vi "Simple SFTP File Download.vi"() -> ()   [LabVIEW 2018]
doc: "Downloads, or receives, a relatively small file from a remote SFTP server. This is similar to the SFTP command line utility when transferring, or copying, a remote file to a local destination. If performance is poor or memory is limited on the local machine, then it could be because the file is relatively large and this implementation is not very efficient for relatively large files."
uses:
  Toolkit/Session/Support/Create from SSH.vi
  Toolkit/Session/Support/Password Authentication.vi
  Toolkit/SFTP/Support/Create from Session.vi
  Toolkit/SFTP File/Support/Open from SFTP.vi
  Toolkit/SFTP File/Support/Close to SFTP.vi
  Toolkit/SFTP/Support/Destroy to Session.vi
  Toolkit/Session/Support/Destroy to SSH.vi
  Toolkit/SSH/SSH.lvclass
  Toolkit/Session/Session.lvclass
  Toolkit/SFTP/SFTP.lvclass
  Toolkit/SFTP File/SFTP File.lvclass
panel:
  in  "Remote File":string
  in  "Local File":path
  in  "Remote SFTP Server":string
  in  "Password":string
  in  "Username":string
  # "Overview: Demonstrates transferring, or downloading, a remote file from a SSH server, similar to the SFTP command line utility\nInstructions:\n1. Enter the IP address or host name of the remote SFTP server. This can be a CompactRIO (cRIO) running the National Instruments Linux Real-Time (NI Linux RT) operating system with the Enable Secure Shell Server (sshd) checkbox checked. \n2. Enter a username. If using a cRIO with a default configuration, then the username is \"admin\".\n3. Enter a password for the username. If using a cRIO with a default configuration, then the password is blank (empty).\n4. Enter the path and/or filename of the remote file to download. Typically, this is a POSIX/UNIX file path with a backslash, \"/\", used to separate directories and the default directory is the remote user's home directory, i.e. \"/home/admin\" on a default configured cRIO.\n5. Select a destination on the local computer for the transfer/download from the remote SSH server.\n6. Run this VI."
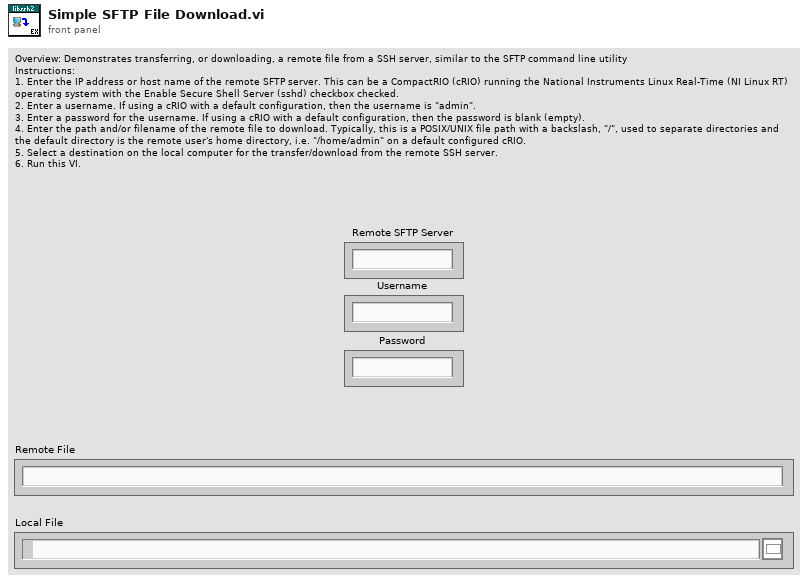
[diagram p1: front panel]
types:
  T1 = enum16{"open", "replace", "create", "open or create", "replace or create", "replace or create with confirmation"}
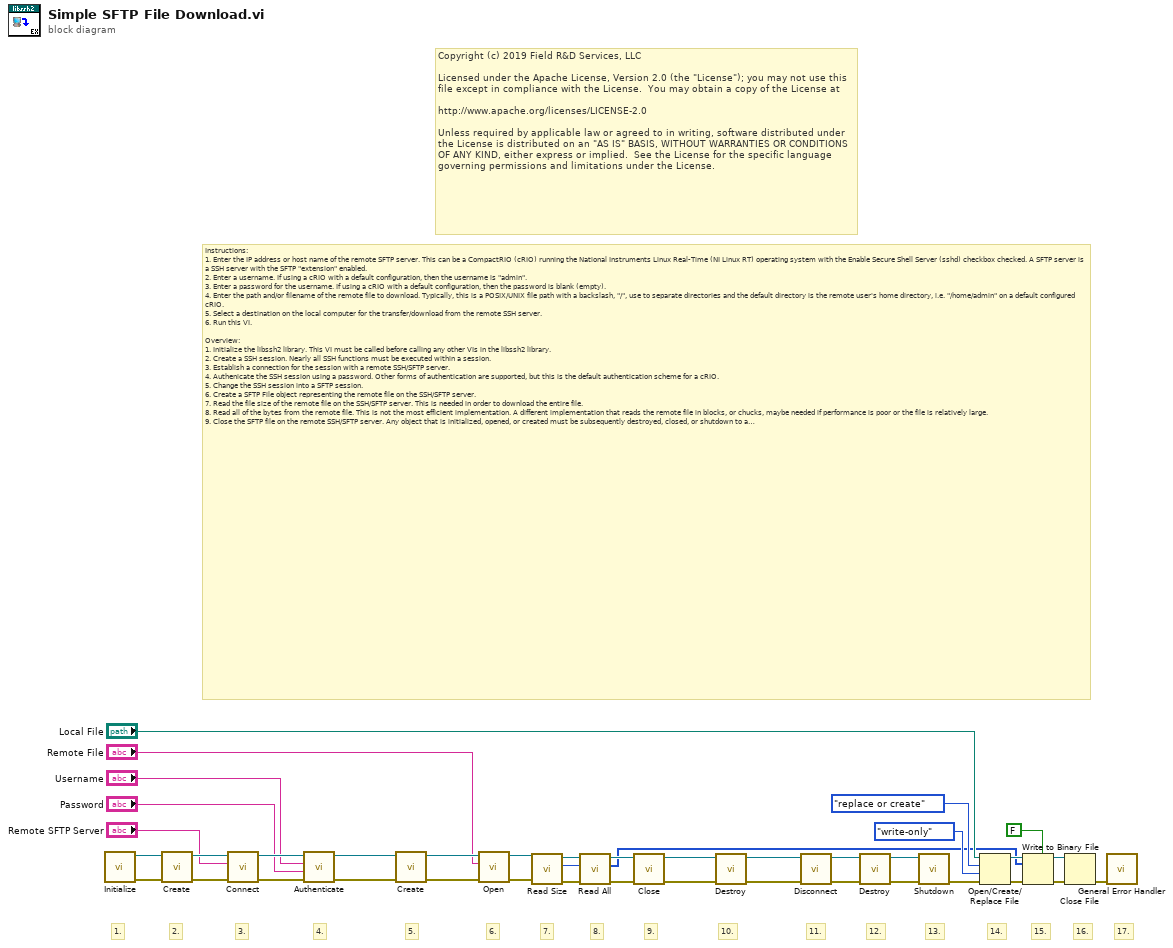
[diagram p0: block diagram]
diagram:
  # "8."
  # "17."
  # "16."
  # "Copyright (c) 2019 Field R&D Services, LLC\n\nLicensed under the Apache License, Version 2.0 (the \"License\"); you may not use this file except in compliance with the License.  You may obtain a copy of the License at\n\nhttp://www.apache.org/licenses/LICENSE-2.0\n\nUnless required by applicable law or agreed to in writing, software distributed under the License is distributed on an \"AS IS\" BASIS, WITHOUT WARRANTIES OR CONDITIONS OF ANY KIND, either express or implied.  See the License for the specific language governing permissions and limitations under the License."
  # "15."
  # "14."
  # "13."
  # "12."
  # "11."
  # "10."
  # "9."
  # "7."
  # "6."
  # "5."
  # "4."
  # "3."
  # "2."
  # "1."
  # "Instructions:\n1. Enter the IP address or host name of the remote SFTP server. This can be a CompactRIO (cRIO) running the National Instruments Linux Real-Time (NI Linux RT) operating system with the Enable Secure Shell Server (sshd) checkbox checked. A SFTP server is a SSH server with the SFTP \"extension\" enabled.\n2. Enter a username. If using a cRIO with a default configuration, then the username is \"admin\".\n3. Enter a password for the username. If using a cRIO with a default configuration, then the password is blank (empty).\n4. Enter the path and/or filename of the remote file to download. Typically, this is a POSIX/UNIX file path with a backslash, \"/\", use to separate directories and the default directory is the remote user's home directory, i.e. \"/home/admin\" on a default configured cRIO.\n5. Select a destination on the local computer for the transfer/download from the remote SSH server.\n6. Run this VI.\n\nOverview:\n1. Initialize the libssh2 library. This VI must be called before calling any other VIs in the libssh2 library.\n2. Create a SSH session. Nearly all SSH functions must be executed within a session.\n3. Establish a connection for the session with a remote SSH/SFTP server.\n4. Authenicate the SSH session using a password. Other forms of authentication are supported, but this is the default authentication scheme for a cRIO. \n5. Change the SSH session into a SFTP session.\n6. Create a SFTP File object representing the remote file on the SSH/SFTP server.\n7. Read the file size of the remote file on the SSH/SFTP server. This is needed in order to download the entire file.\n8. Read all of the bytes from the remote file. This is not the most efficient implementation. A different implementation that reads the remote file in blocks, or chucks, maybe needed if performance is poor or the file is relatively large.\n9. Close the SFTP file on the remote SSH/SFTP server. Any object that is initialized, opened, or created must be subsequently destroyed, closed, or shutdown to avoid memory leaks, undefined behavior, or crashes.\n10. Change the SFTP session back into a SSH session.\n11. Disconnect from the remote SSH server.\n12. Destroy the session to free resources within the libssh2 library.\n13. Shutdown the libssh2 library. This VI must be last VI called for the libssh2 library. No other libssh2 VIs should be called once this VI is executed.\n14. Create or replace (overwrite) a file to write the read contents from the remote file.\n15. Write the data from the remote file.\n16. Close the file. This is not strictly necessary, but it is good practice.\n19. Provide some error handling and reporting. Libssh2 errors will be in the -8100 range."
  n1 = call "Initialize.vi"() -> ("Error Out"=w29:errorcluster, "SSH"=w28:refnum<class "SSH.lvclass">)  [unwired: 10 in]
  n2 = call-poly "Create.vi"("Error In"=w29, "SSH"=w28) -> ("Error Out"=w39:errorcluster, "Sesssion"=w40:refnum<class "Session.lvclass">)  [unwired: 8 in]
  n3 = call "Connect.vi"("Error In"=w39, "Address"="Remote SFTP Server", "Session In"=w40) -> ("Error Out"=w37:errorcluster, "Sesssion Out"=w38:refnum<class "Session.lvclass">)  [unwired: 7 in]
  n4 = call-poly "Authenticate.vi"("Error In"=w37, "Password"="Password", "Username"="Username", "Session In"=w38) -> ("Error Out"=w17:errorcluster, "Sesssion Out"=w18:refnum<class "Session.lvclass">)  [unwired: 6 in]
  n5 = call-poly "Create.vi"("Error In"=w17, "Session"=w18) -> ("Error Out"=w15:errorcluster, "SFTP"=w16:refnum<class "SFTP.lvclass">)  [unwired: 8 in]
  n6 = call-poly "Open.vi"("Error In"=w15, "Remote Path"="Remote File", "SFTP"=w16) -> ("Error Out"=w3:errorcluster, "SFTP File"=w4:refnum<class "SFTP File.lvclass">)  [unwired: 7 in]
  n7 = call "Read Size.vi"("Error In"=w3, "SFTP File In"=w4) -> ("Error Out"=w1:errorcluster, "File Size"=w5:u64, "SFTP File Out"=w2:refnum<class "SFTP File.lvclass">)  [unwired: 7 in]
  n8 = call "Read All.vi"("Error In"=w1, "Max Read Size"=w5, "SFTP File In"=w2) -> ("Error Out"=w8:errorcluster, "Data"=w7:u8[], "SFTP File Out"=w9:refnum<class "SFTP File.lvclass">)  [unwired: 6 in]
  n9 = call-poly "Close.vi"("Error In"=w8, "SFTP File"=w9) -> ("Error Out"=w12:errorcluster, "SFTP"=w13:refnum<class "SFTP.lvclass">)  [unwired: 7 in, 1 out]
  n10 = call-poly "Destroy.vi"("Error In"=w12, "SFTP"=w13) -> ("Error Out"=w10:errorcluster, "Session"=w11:refnum<class "Session.lvclass">)  [unwired: 8 in]
  n11 = call "Disconnect.vi"("Error In"=w10, "Session In"=w11) -> ("Error Out"=w32:errorcluster, "Sesssion Out"=w33:refnum<class "Session.lvclass">)  [unwired: 8 in]
  n12 = call-poly "Destroy.vi"("Error In"=w32, "Session"=w33) -> ("Error Out"=w30:errorcluster, "SSH"=w31:refnum<class "SSH.lvclass">)  [unwired: 8 in]
  n13 = call "Shutdown.vi"("Error In"=w30, "SSH"=w31) -> ("Error Out"=w27:errorcluster)  [unwired: 9 in]
  n14 = Open/Create/Replace File(file path (use dialog)="Local File", error in=w27, operation (0:open)=T1."replace or create", access (0:read/write)=enum16{"read/write", "read-only", "write-only"}."write-only") -> (refnum out=w23:refnum<file>, error out=w22:errorcluster)  [unwired: 2 in, 1 out]
  n15 = Write to Binary File(file (use dialog)=w23, data=w7, error in=w22, 5:FALSE ("prepend array or string size? (T)")) -> (refnum out=w21:refnum<file>, error out=w20:errorcluster)  [unwired: 2 in, 1 out]
  n16 = Close File(refnum=w21, error in=w20) -> (error out=w19:errorcluster)  [unwired: 1 out]
  n17 = call <vilib>:"General Error Handler.vi"("error in (no error)"=w19) -> ()  [unwired: 10 in, 5 out]
